vi "VIH Project Tree - Add File Group.vi"(8 "error in":errorcluster, 9 "Group Name":string, 10 "Tree Parent Tag":string, 11 "Project Tree":T1) -> (0 "error out":errorcluster, 1 "Item Tag":string, 2 "dup Tree Parent Tag":string, 3 "dup Project Tree":T1)   [LabVIEW 2014]
doc: "::: VI Helpeks :::\nCopyright (c) 2000-2026 Konstantin Shifershteyn. All rights reserved."
uses:
  VIH Project Tree Typedef - Tree Refnum.ctl
  VIH Project Tree Typedef - Tree Item Type.ctl
panel:
  # "VI Helpeks\nCopyright (c) 2012-2026 Konstantin Shifershteyn"
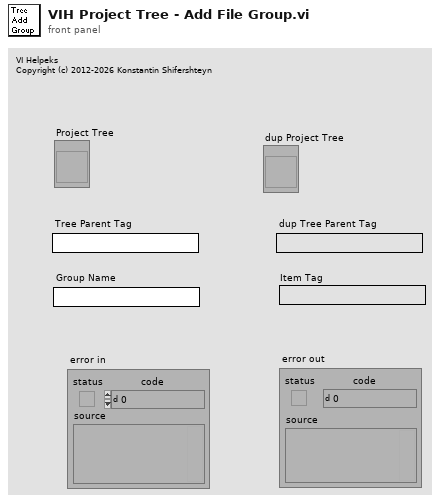
[diagram p1: front panel]
types:
  T1 = typedef "VIH Project Tree Typedef - Tree Refnum.ctl" = refnum<vi>
  T2 = typedef "VIH Project Tree Typedef - Tree Item Type.ctl" = enum32{"<Invalid>", "Project", "Proj Files", "Proj Rules", "File Group", "Rule Group", "Any File", "LV Func", ".mnu", ".mnu (dyn)", ".vi", ".vi (dyn)", ".vit", ".vit (dyn)", ".ctl", ".ctl (dyn)", ".ctt", ".ctt (dyn)", "polyVI", "polyVI (dyn)", "expVI", "expVI (dyn)", "HTML", "PolyVI Inst"}
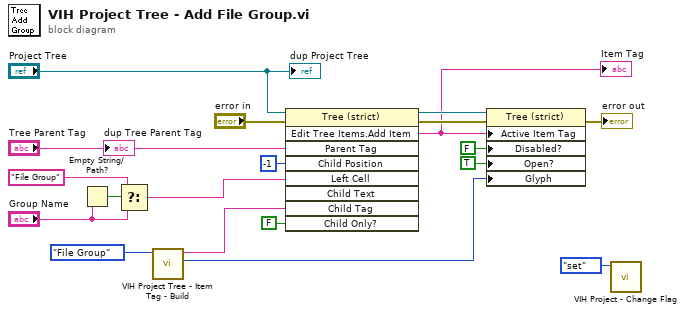
[diagram p0: block diagram]
diagram:
  n1 = Empty String/Path?(string/path="Group Name") -> (empty?=w14:bool)
  n2 = Select(t="File Group" ("Left Cell String"), s=w14, f="Group Name") -> (s? t:f=w12:string)
  n3 = call "VIH Project Tree - Item Tag - Build.vi"("Item Type"=VIH_Project_Tree_Typedef_-_Tree_Item_Type."File Group") -> ("Tree Item Symbol"=w3:i32, "Tree Item Tag"=w5:string)  [unwired: 9 in]
  n4 = invoke on="Invoke Node" class="Tree (strict)" method="Edit Tree Items.Add Item"(reference="Project Tree", error in="error in", "Parent Tag"="Tree Parent Tag", "Child Position"=-1, "Left Cell"=w12, "Child Tag"=w5, "Child Only?"=FALSE) -> (reference out=w19:T1, error out=w9:errorcluster, "Edit Tree Items:Add Item"=w6:string)  [unwired: 2 in, 6 out]
  "Item Tag" <- w6
  n5 = property on="Property Node" class="Tree (strict)"(reference=w19, error in=w9, "Active Item Tag"=w6, "Disabled?"=FALSE ("Active Item:Disabled?"), "Open?"=TRUE ("Active Item:Open?"), "Glyph"=w3) -> (error out=→"error out":errorcluster)  [unwired: 1 out]
  n6 = call "VIH Project - Change Flag.vi"("cmd (get)"=enum16{"get", "set", "reset"}."set") -> ()  [unwired: 9 in, 2 out]
  "dup Project Tree" <- "Project Tree"
  "dup Tree Parent Tag" <- "Tree Parent Tag"
